vi "collision detection.vi"(7 "y values 2":dbl[](array[numeric]), 8 "error in (no error)":errorcluster, 9 "x values":dbl[](array[numeric]), 10 "x values 2":dbl[](array[numeric]), 11 "y values":dbl[](array[numeric])) -> (0 "error out":errorcluster, 3 "Collision":bool)   [LabVIEW 2018]
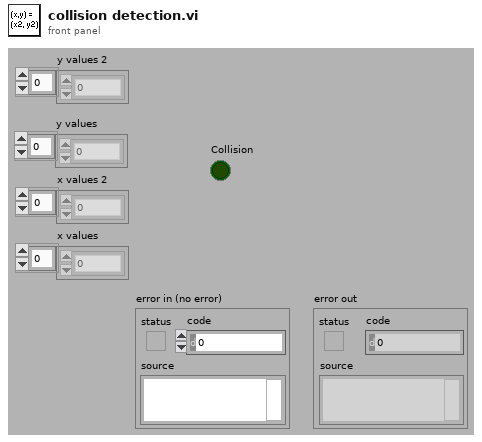
[diagram p1: front panel]
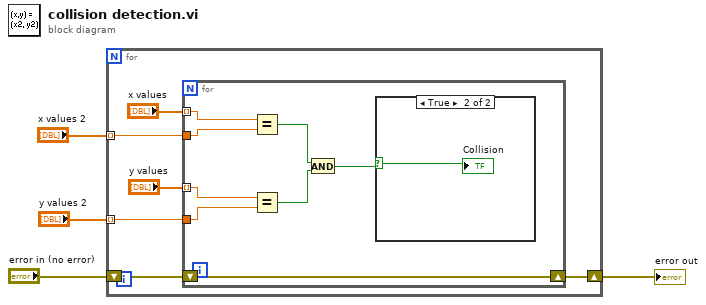
[diagram p0: block diagram]
diagram:
  n1 = for {
    shift-right: [w5] -> w1
    shift-left: "error in (no error)" -> [w6]
    tunnel: "x values 2" -> [w9] mode=indexing
    tunnel: "y values 2" -> [w8] mode=indexing
    n2 = for {
      tunnel: "x values" -> [w18] mode=indexing
      tunnel: w9 -> [w17]
      tunnel: w8 -> [w15]
      tunnel: "y values" -> [w16] mode=indexing
      shift-right: [w14] -> w5
      shift-left: w6 -> [w14]
      n3 = Equal?(x=w18, y=w17) -> (x = y?=w12:bool)
      n4 = Equal?(x=w16, y=w15) -> (x = y?=w13:bool)
      n5 = And(x=w12, y=w13) -> (x .and. y?=w11:bool)
      n6 = case shown="True" w11 {
        selector: w11 -> [_ w19]
        frame False {
        }
        frame True {
          "Collision" <- w19
        }
      }
    }
  }
  "error out" <- w1
